vi "Correlation_Contrast.vi"() -> ()   [LabVIEW 2024]
uses:
  Global_Stop.vi
panel:
  in  "Tau Step Size":dbl=2.5e-07
  out "Current Tau":dbl
  in  "N":dbl=5.0
  out "XY Graph":cluster{"Y":dbl[], "Y":dbl[]}[](graph)
  out "At step":i32
  out "data":dbl[](array[numeric])
  out "B Gate":dbl[][](array[numeric])
  out "A Gate":dbl[][](array[numeric])
  out "DATA":dbl[][](array[numeric])
  in  "stop":bool
  in  "Number of steps":i32=200
  out "At pass":i32
  in  "Number of individual passes?":i32=50
  in  "Frequency in MHz":string="f2585"
  in  "file path (use dialog)":path=path "C:/Users/Crawford Group/Desktop/DATA (labVIEW Writes)/Coralation Contrast/B Gate.txt"
  in  "file path (use dialog) 2":path=path "C:/Users/Crawford Group/Desktop/DATA (labVIEW Writes)/Coralation Contrast/A Gate.txt"
  in  "file path (use dialog) 3":path=path "C:/Users/Crawford Group/Desktop/DATA (labVIEW Writes)/Coralation Contrast/Average.txt"
  in  "T set":string="9E3"
  in  "A Gate Delay":dbl=0.0001177
  in  "B Gate Delay":dbl=243.4
  in  "Use gate delay commands?":bool=TRUE
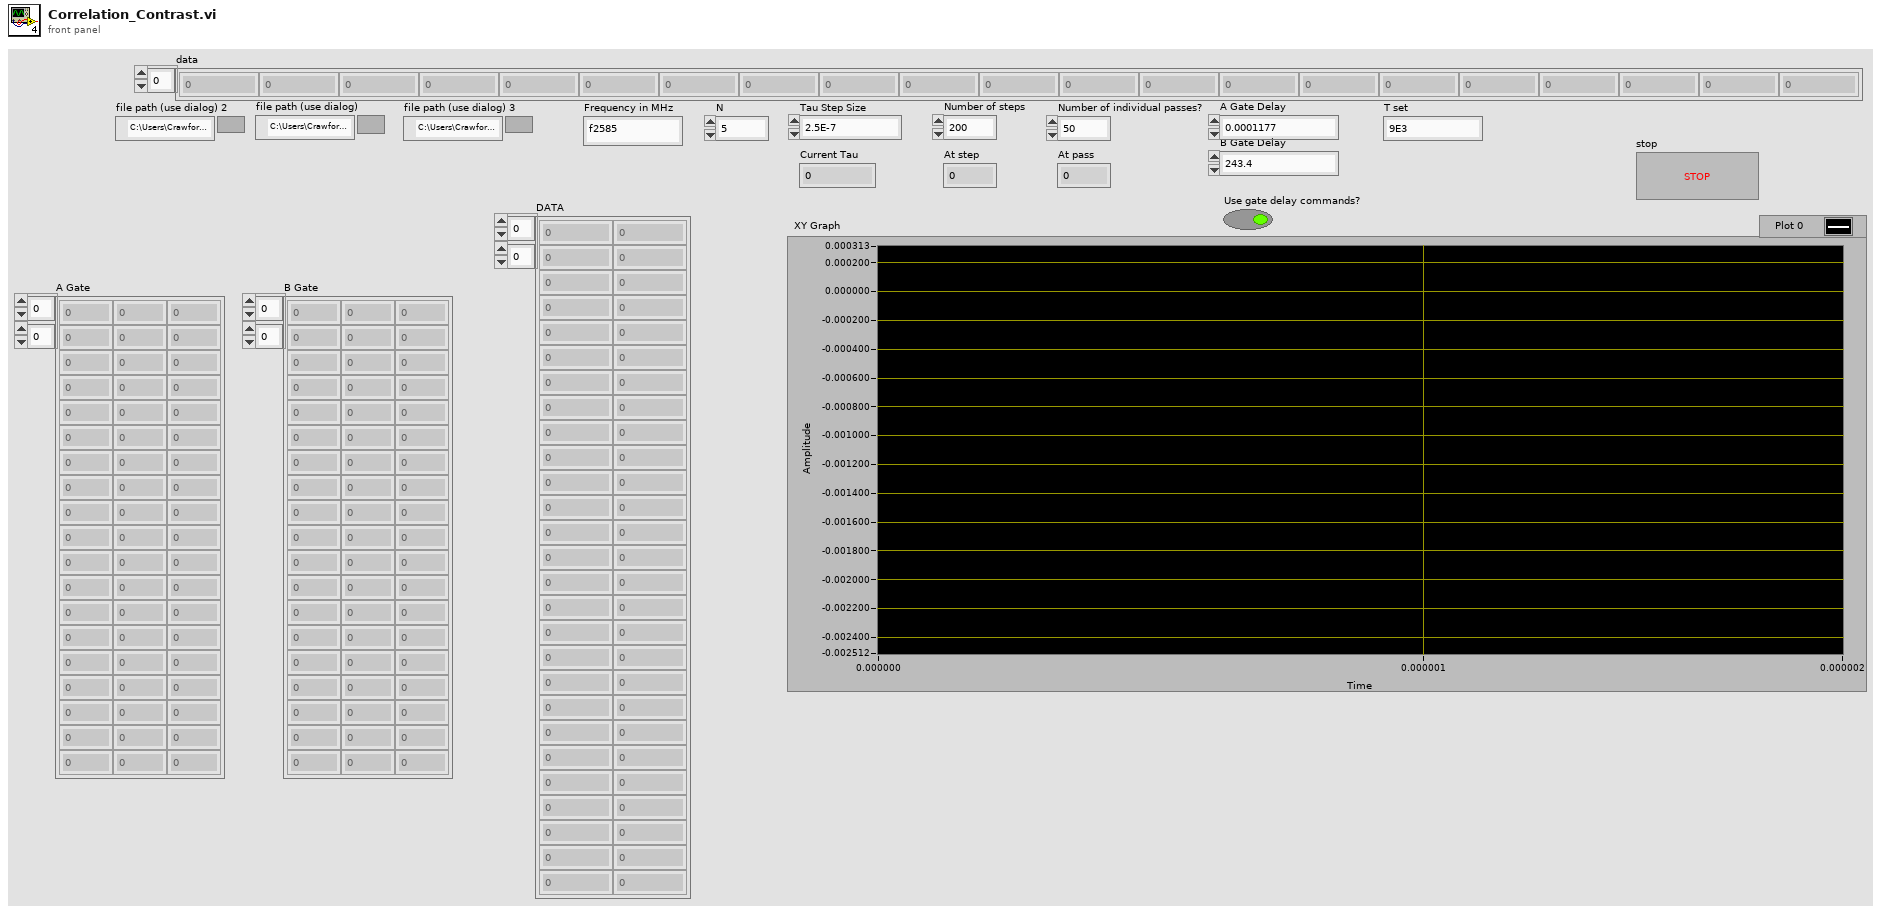
[diagram p1: front panel]
types:
  T1 = enum16{"open", "replace", "create", "open or create", "replace or create", "replace or create with confirmation"}
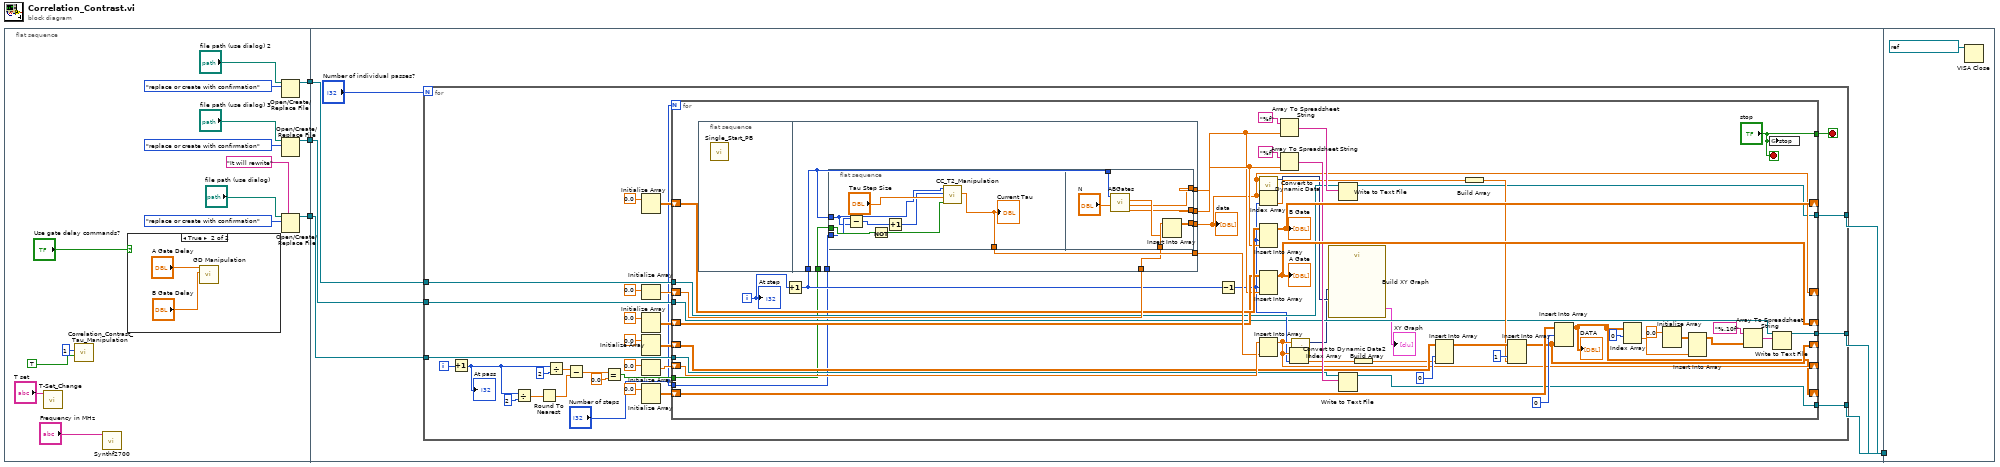
[diagram p0: block diagram]
diagram:
  n1 = flat-sequence {
    tunnel: [w17] -> w6
    tunnel: [w14] -> w5
    tunnel: [w11] -> w4
    tunnel: w6 -> [w30]
    tunnel: w5 -> [w29]
    tunnel: w4 -> [w28]
    tunnel: [w27] -> w3
    tunnel: [w26] -> w2
    tunnel: [w25] -> w1
    tunnel: w3 -> [_]
    tunnel: w2 -> [_]
    tunnel: w1 -> [_]
    frame #0 {
      n2 = call "T-Set_Change.vi"("T set"="T set") -> ()  [unwired: 11 in]
      n3 = call "Correlation_Contrast_Tau_Manipulation.vi"("Dont invert?"=TRUE ("Invert?"), "Numeric"=1) -> ()  [unwired: 9 in, 1 out]
      n4 = call "Synthf2700.vi"("Frequency in MHz"="Frequency in MHz") -> ()  [unwired: 11 in]
      n5 = case shown="True" "Use gate delay commands?" {
        frame False {
        }
        frame True {
          n6 = call "GD Manipulation.vi"("B Gate delay"="B Gate Delay", "A Gate Delay"="A Gate Delay") -> ()  [unwired: 10 in]
        }
      }
      n7 = Open/Create/Replace File(file path (use dialog)="file path (use dialog) 2", operation (0:open)=T1."replace or create with confirmation") -> (refnum out=w14:refnum<file>)  [unwired: 4 in, 2 out]
      n8 = Open/Create/Replace File(file path (use dialog)="file path (use dialog) 3", operation (0:open)=T1."replace or create with confirmation") -> (refnum out=w11:refnum<file>)  [unwired: 4 in, 2 out]
      n9 = Open/Create/Replace File(file path (use dialog)="file path (use dialog)", prompt="It will rewrite", operation (0:open)=T1."replace or create with confirmation") -> (refnum out=w17:refnum<file>)  [unwired: 3 in, 2 out]
    }
    frame #1 {
      n10 = for {
        N: "Number of individual passes?" -> [_]
        tunnel: w30 -> [w52]
        tunnel: [w45] -> w27
        tunnel: w28 -> [w46]
        tunnel: [w44] -> w26
        tunnel: w29 -> [w51]
        tunnel: [w43] -> w25
        i -> [w39]
        stop <- w31 stop-if-true
        n11 = Increment(x=w39) -> (x+1=w38:i32)
        "At pass" <- w38
        n12 = Divide(x=w38, y=2) -> (x/y=w35:dbl)
        n13 = Round To Nearest(number=w35) -> (nearest integer value=w34:dbl)
        n14 = Divide(x=w38, y=2) -> (x/y=w40:dbl)
        n15 = Subtract(x=w40, y=w34) -> (x-y=w37:dbl)
        n16 = Equal?(x=w37, y=0.0) -> (x = y?=w33:bool)
        n17 = Initialize Array(0.0) -> (w54:dbl[][])  [unwired: 2 in]
        n18 = Initialize Array(0.0) -> (w60:dbl[])  [unwired: 1 in]
        n19 = Initialize Array(0.0) -> (w53:dbl[][])  [unwired: 2 in]
        n20 = Initialize Array(0.0) -> (w49:dbl[][])  [unwired: 2 in]
        n21 = Initialize Array(0.0) -> (w59:dbl[])  [unwired: 1 in]
        n22 = Initialize Array(0.0) -> (w47:dbl[][])  [unwired: 2 in]
        n23 = for {
          N: "Number of steps" -> [_]
          shift-right: [w82] -> _
          shift-left: w60 -> [w109]
          shift-right: [w87] -> _
          shift-left: w59 -> [w108]
          shift-right: [w103] -> _
          shift-left: w54 -> [w106]
          shift-right: [w104] -> _
          shift-left: w53 -> [w105]
          tunnel: w52 -> [w101]
          tunnel: w51 -> [w97]
          shift-right: [w74] -> _
          shift-left: w49 -> [w91]
          shift-right: [w70] -> _
          shift-left: w47 -> [w90]
          tunnel: w46 -> [w78]
          tunnel: [w69] -> w45
          tunnel: [w68] -> w44
          tunnel: [w67] -> w43
          tunnel: w33 -> [w65]
          tunnel: "Number of steps" -> [w64]
          tunnel: ["stop"] -> w31
          i -> [w66]
          stop <- "stop" stop-if-true
          n24 = flat-sequence {
            tunnel: w88 -> [w114]
            tunnel: w109 -> [w113]
            tunnel: [w112] -> w82
            tunnel: [w117] -> w107
            tunnel: [w110] -> w96
            tunnel: [w111] -> w99
            tunnel: w65 -> [w116]
            tunnel: w64 -> [w115]
            frame #0 {
              n25 = call "Single_Start_PB.vi"() -> ()  [unwired: 12 in]
            }
            frame #1 {
              n26 = flat-sequence {
                tunnel: w114 -> [w118]
                tunnel: [w122] -> w117
                tunnel: w116 -> [w125]
                tunnel: w115 -> [w124]
                tunnel: w114 -> [w131]
                tunnel: w113 -> [w130]
                tunnel: [w128] -> w112
                tunnel: [w127] -> w111
                tunnel: [w126] -> w110
                frame #0 {
                  n27 = Subtract(x=w124, y=w118) -> (x-y=w123:i32)
                  n28 = Not(x=w125) -> (.not. x?=w121:bool)
                  n29 = Increment(x=w123) -> (x+1=w119:i32)
                  n30 = call "CC_T2_Manipulation.vi"("Invert?"=w121, "Tau Step Size"="Tau Step Size", "Numeric 2"=w119, "Numeric"=w118) -> ("Tau"=w122:dbl)  [unwired: 7 in]
                  "Current Tau" <- w122
                }
                frame #1 {
                  n31 = call "ABGates.vi"("N"="N", "# of loop"=w131) -> ("B Gate"=w127:dbl[], "A Gate"=w126:dbl[], "average A-B/A+B"=w129:dbl)  [unwired: 7 in]
                  n32 = Insert Into Array(array=w130, new element=w129) -> (w128:dbl[])  [unwired: 1 in]
                }
              }
            }
          }
          n33 = Increment(x=w66) -> (x+1=w88:i32)
          n34 = Decrement(x=w88) -> (x-1=w81:i32)
          n35 = call "Convert to Dynamic Data"("Array"=w82) -> ("Dynamic Data Type"=w62:dynamicdata)  [unwired: 3 in]
          n36 = Index Array(array=w82, index=w81) -> (element=w84:dbl)
          n37 = Insert Into Array(array=w106, index (col)=w81, new element=w99) -> (w103:dbl[][])  [unwired: 1 in]
          "B Gate" <- w103
          n38 = Insert Into Array(array=w105, index (col)=w81, new element=w96) -> (w104:dbl[][])  [unwired: 1 in]
          "A Gate" <- w104
          n39 = Insert Into Array(array=w108, new element=w107) -> (w87:dbl[])  [unwired: 1 in]
          n40 = Array To Spreadsheet String(array=w96, 3:"%f" ("format string")) -> (spreadsheet string=w98:string)  [unwired: 1 in]
          n41 = Array To Spreadsheet String(array=w99, 3:"%f" ("format string")) -> (spreadsheet string=w102:string)  [unwired: 1 in]
          n42 = Index Array(array=w87, index=w81) -> (element=w86:dbl)
          n43 = call "Convert to Dynamic Data2"("Array"=w87) -> ("Dynamic Data Type"=w61:dynamicdata)  [unwired: 3 in]
          n44 = call "Build XY Graph"("Y Input"=w62, "X Input"=w61) -> ("XY Graph"=→"XY Graph":cluster{"X":dbl[], "Y":dbl[]}[])  [unwired: 8 in, 1 out]
          n45 = Write to Text File(file (use dialog)=w97, text=w98) -> (refnum out=w68:refnum<file>)  [unwired: 2 in, 2 out]
          n46 = Write to Text File(file (use dialog)=w101, text=w102) -> (refnum out=w69:refnum<file>)  [unwired: 2 in, 2 out]
          n47 = Build Array(w86) -> (w85:dbl[])
          n48 = Insert Into Array "Insert Into Array"(array=w91, index (col)=0 ("disabled index (col)"), new element=w85) -> (w92:dbl[][])  [unwired: 1 in]
          n49 = Build Array(w84) -> (w83:dbl[])
          n50 = Insert Into Array(array=w92, index (col)=1 ("disabled index (col)"), new element=w83) -> (w74:dbl[][])  [unwired: 1 in]
          n51 = Insert Into Array(array=w90, index (row)=0, new element=w74) -> (w70:dbl[][])  [unwired: 1 in]
          "DATA" <- w70
          n52 = Index Array(array=w70, index (row)=0) -> (element=w72:dbl[])  [unwired: 1 in]
          n53 = Initialize Array(0.0 ("element")) -> (w71:dbl[][])  [unwired: 2 in]
          n54 = Insert Into Array(array=w71, new element=w72) -> (w75:dbl[][])  [unwired: 2 in]
          n55 = Array To Spreadsheet String(array=w75, 3:"%.10f" ("format string")) -> (spreadsheet string=w79:string)  [unwired: 1 in]
          n56 = global write "Global_Stop.vi" "stop"("stop") -> ()
          n57 = Write to Text File(file (use dialog)=w78, text=w79) -> (refnum out=w67:refnum<file>)  [unwired: 2 in, 2 out]
          "At step" <- w66
          "data" <- w82
        }
      }
    }
    frame #2 {
      n58 = VISA Close(VISA resource name=refnum<visa-resource-name> "GPIB0::23::INSTR") -> ()  [unwired: 1 in, 1 out]
    }
  }
